vi "User Events Metadata.vi"(8 "error in":errorcluster, 10 "Reply Payload":T1 {"Replay Metadata"."Relative seconds (Frame 0)" format="%#_13g"; "Replay Metadata"."Relative seconds (User Event)" format="%#_13g"}) -> (0 "error out":errorcluster)   [LabVIEW 2026, in "Replay.lvlib"]
doc: "_____\nCreated using DQMH Framework: Event Scripter 7.1.2.1547."
uses:
  Replay.lvlib
  Load UserEvents (Reply Payload)--cluster.ctl
  User Events Metadata.ctl
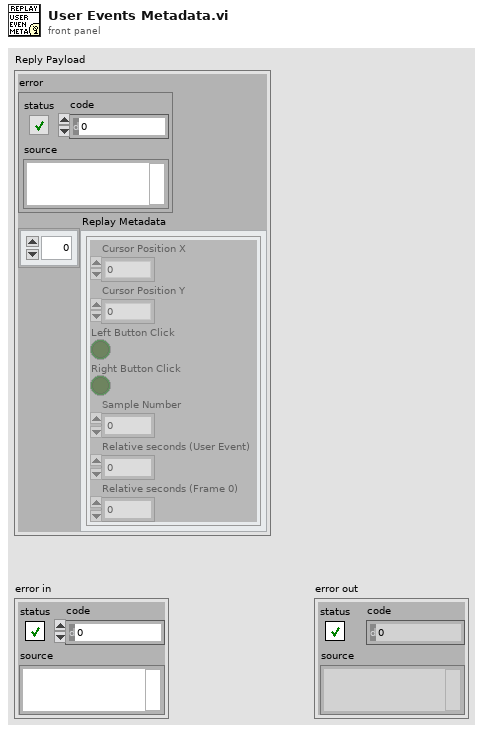
[diagram p1: front panel]
types:
  T1 = typedef "Replay.lvlib/Load UserEvents (Reply Payload)--cluster.ctl" = cluster{"error":errorcluster, "Replay Metadata":T2[]}
  T2 = typedef "User Events Metadata.ctl" = cluster{"Cursor Position X":i32, "Cursor Position Y":i32, "Left Button Click":bool, "Right Button Click":bool, "Sample Number":u32, "Relative seconds (User Event)":dbl, "Relative seconds (Frame 0)":dbl}
  T3 = typedef "Replay.lvlib/Broadcast Events--cluster.ctl" = cluster{"Module Did Init":refnum<user-event>, "Status Updated":refnum<user-event>, "Error Reported":refnum<user-event>, "Module Did Stop":refnum<user-event>, "Update Module Execution Status":refnum<user-event>, "Replay Finished Processing User Events":refnum<user-event>, "User Events Metadata":refnum<user-event>}
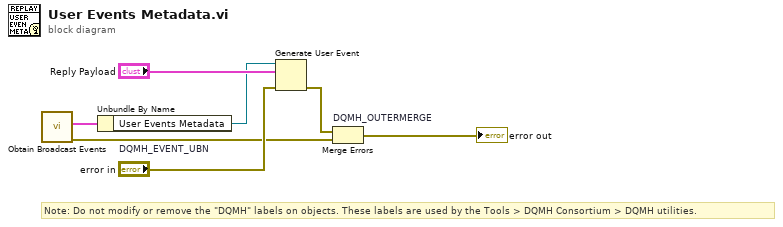
[diagram p0: block diagram]
diagram:
  # "Note: Do not modify or remove the \"DQMH\" labels on objects. These labels are used by the Tools > DQMH Consortium > DQMH utilities."
  n1 = call "Obtain Broadcast Events.vi"() -> ("error out"=w2:errorcluster, "Replay Broadcast Events"=w1:T3)  [unwired: 10 in]
  n2 = Unbundle By Name "DQMH_EVENT_UBN"(w1) -> ("User Events Metadata"=w4:refnum<user-event>)
  n3 = Generate User Event(user event=w4, event data cluster="Reply Payload", error in="error in") -> (error out=w3:errorcluster)  [unwired: 1 in, 1 out]
  n4 = Merge Errors "DQMH_OUTERMERGE"(w3, w2) -> (→"error out":errorcluster)
